vi "Disconnect.vi"(8 "error in (no error)":errorcluster, 11 "object in":refnum<class "AIO_Channel.lvclass">) -> (0 "error out":errorcluster, 3 "object out":refnum<class "AIO_Channel.lvclass">)   [LabVIEW 2021, in "DAQmx.lvlib" / "AIO_Channel.lvclass"]
uses:
  AIO_Channel.lvclass
  AIO_Channel.lvclass/AIO_Channel.ctl
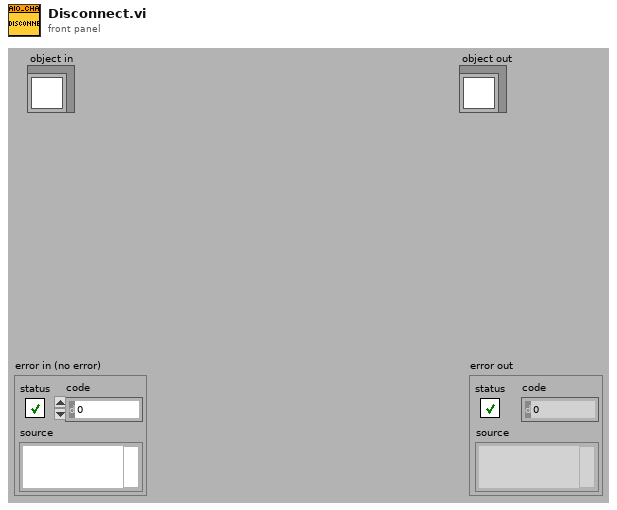
[diagram p1: front panel]
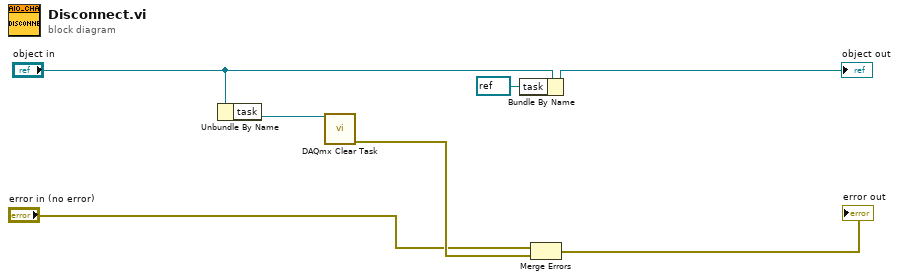
[diagram p0: block diagram]
diagram:
  n1 = Unbundle By Name("object in") -> ("task"=w5:refnum<k21>)
  n2 = call <vilib>:"DAQmx Clear Task.vi"("task in"=w5) -> ("error out"=w7:errorcluster)  [unwired: 14 in]
  n3 = Bundle By Name(cluster="object in", "task"=refnum<k21> refnum) -> (→"object out":refnum<class "AIO_Channel.lvclass">)
  n4 = Merge Errors("error in (no error)", w7) -> (→"error out":errorcluster)
